vi "Change TeraTerm Ant Pol.vi"(8 "error in (no error)":errorcluster caption="에러 입력(에러 없음)", 10 "Antenna Pol":enum16{"H", "V"}(ring), 11 "Instrument Manager 입력":refnum<class "Instrument Manager.lvclass">) -> (0 "error out":errorcluster caption="에러 출력", 3 "Instrument Manager 출력":refnum<class "Instrument Manager.lvclass">)   [LabVIEW 2023, in "Instrument Manager.lvclass"]
uses:
  Instrument Manager.lvclass
  Instrument Manager.lvclass/Instrument Manager.ctl
panel:
  out "Success?":bool
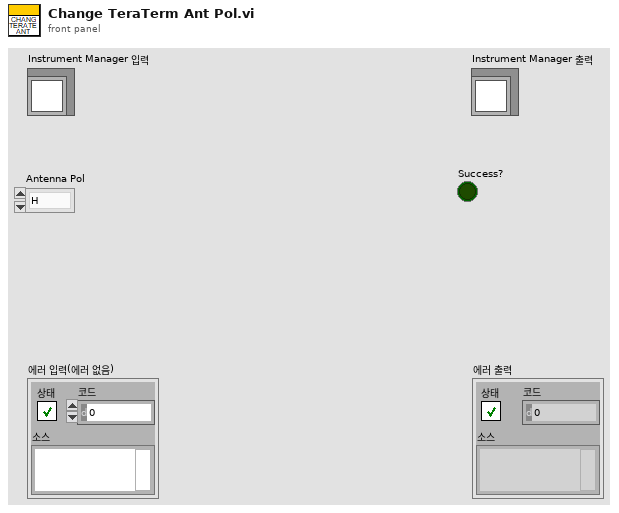
[diagram p1: front panel]
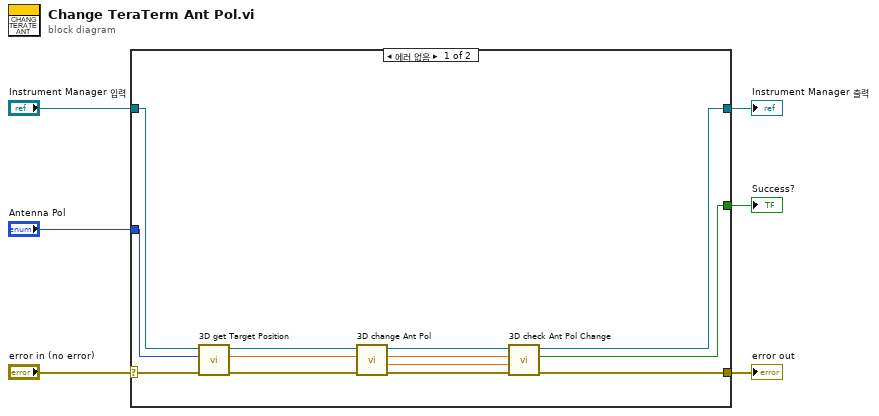
[diagram p0: block diagram]
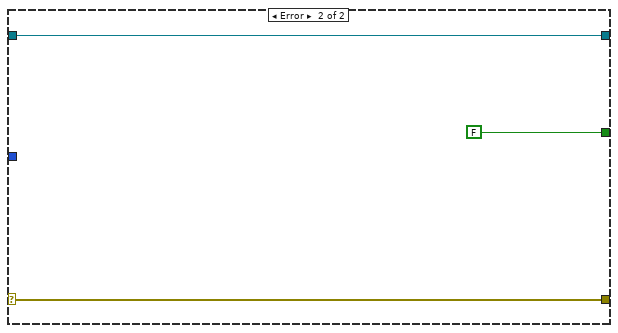
[diagram p2: hidden frame]
diagram:
  n1 = case shown="에러 없음" "error in (no error)" {
    selector: "error in (no error)" -> [w18 w21]
    tunnel: [w9 w21] -> w5
    tunnel: [w8 w20] -> w3
    tunnel: "Instrument Manager 입력" -> [w17 w20]
    tunnel: "Antenna Pol" -> [w16 _]
    tunnel: [w7 FALSE ("불리언")] -> w1
    frame No Error {
      n2 = call "3D get Target Position.vi"("error in (no error)"=w18, "Antenna Pol"=w16, "Instrument Manager 입력"=w17) -> ("error out"=w14:errorcluster, "Target Position (deg)"=w13:dbl, "Instrument Manager 출력"=w15:refnum<class "Instrument Manager.lvclass">)  [unwired: 6 in]
      n3 = call "3D change Ant Pol.vi"("error in (no error)"=w14, "Target Position (deg)"=w13, "Instrument Manager 입력"=w15) -> ("error out"=w10:errorcluster, "Current Position (degree)"=w12:dbl, "Instrument Manager 출력"=w11:refnum<class "Instrument Manager.lvclass">)  [unwired: 5 in]
      n4 = call "3D check Ant Pol Change.vi"("error in (no error)"=w10, "Current Position (degree)"=w12, "Target Position (deg)"=w13, "Instrument Manager 입력"=w11) -> ("error out"=w9:errorcluster, "불리언"=w7:bool, "Instrument Manager 출력"=w8:refnum<class "Instrument Manager.lvclass">)  [unwired: 5 in]
    }
    frame Error {
    }
  }
  "error out" <- w5
  "Instrument Manager 출력" <- w3
  "Success?" <- w1
